vi "Configure Displays.vi"(5 "Feedback Chart":refnum<vi>, 7 "Verdict Display":refnum<vi>, 8 "error in":errorcluster, 9 "Channel Values Display":refnum<vi>, 10 "Step Table Display":refnum<vi>, 11 "Sequence Executor in":refnum<class "Sequence Executor.lvclass">) -> (0 "error out":errorcluster, 3 "Sequence Executor out":refnum<class "Sequence Executor.lvclass">)   [LabVIEW 2026, in "Sequence Executor.lvclass"]
doc: "Stores the Step Table Display, Channel Values Display, Verdict Display and Feedback Chart in the actor's private data. Called by the launcher BEFORE Launch Root Actor. Static, public."
uses:
  C:/Users/DynaAdmin/PycharmProjects/Universal-sequence-executor-AF/src/Executor/Sequence Executor.lvclass
  C:/Users/DynaAdmin/PycharmProjects/Universal-sequence-executor-AF/src/Executor/Sequence Executor.lvclass/Sequence Executor.ctl
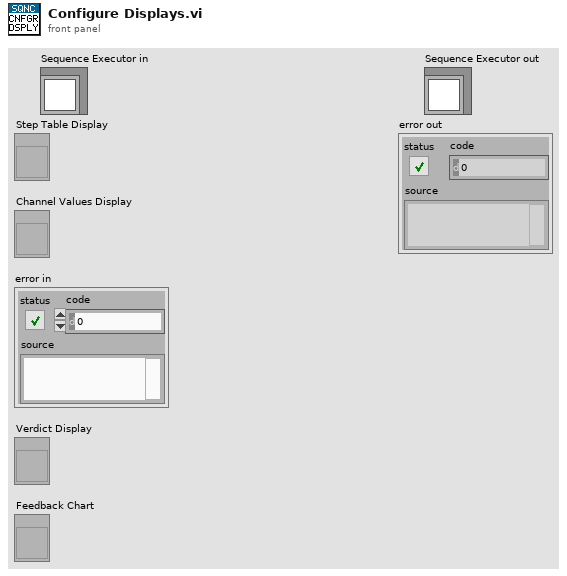
[diagram p1: front panel]
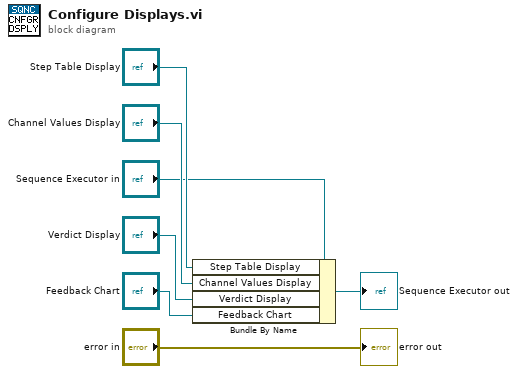
[diagram p0: block diagram]
diagram:
  n1 = Bundle By Name(cluster="Sequence Executor in", "Step Table Display"="Step Table Display", "Channel Values Display"="Channel Values Display", "Verdict Display"="Verdict Display", "Feedback Chart"="Feedback Chart") -> (→"Sequence Executor out":refnum<class "Sequence Executor.lvclass">)
  "error out" <- "error in"
